vi "Save Background.vi"(8 "error in":errorcluster, 10 "File Path":path, 11 "BigMAQ in":refnum<class "BigMAQ.lvclass">) -> (0 "error out":errorcluster, 3 "BigMAQ out":refnum<class "BigMAQ.lvclass">)   [LabVIEW 2019, in "BigMAQ.lvclass"]
uses:
  BigMAQ.lvclass
  BigMAQ.lvclass/BigMAQ.ctl
  <vilib>/LabVIEW Open Source Project/Unicity/RandomStringGenerator/RandomStringGenerator.lvclass
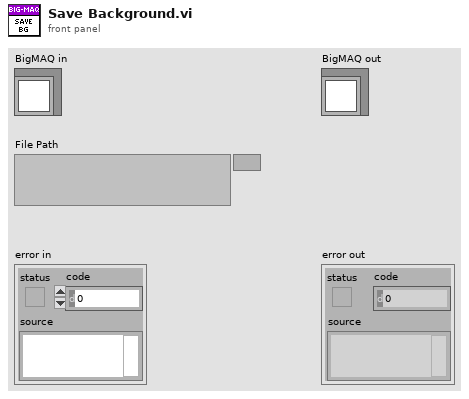
[diagram p1: front panel]
types:
  T1 = typedef "Image Type" = u32
  T2 = typedef "IMAQ Image.ctl" = refnum<image>
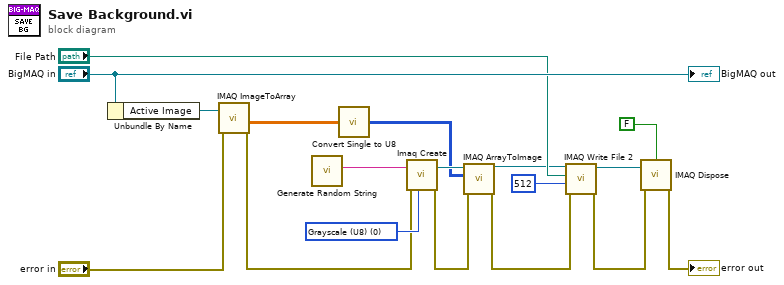
[diagram p0: block diagram]
diagram:
  w12 = T1 0 items=["Grayscale (U8)", "Grayscale (I16)", "Grayscale (SGL)", "Complex (CSG)", "RGB (U32)", "HSL (U32)", "RGB (U64)", "Grayscale (U16)"] ("Image Type")
  n1 = Unbundle By Name("BigMAQ in") -> ("Active Image"=w10:T2)
  n2 = call "IMAQ ImageToArray"("error in (no error)"="error in", "Image"=w10) -> ("Image Pixels (Float)"=w5:sgl[][], "error out"=w2:errorcluster)  [unwired: 2 in, 3 out]
  n3 = call <vilib>:"Generate Random String.vi"() -> ("Random String"=w1:string)  [unwired: 11 in]
  n4 = call "Convert Single to U8.vi"("Image Pixels (Float)"=w5) -> ("Image Pixels (U8)"=w4:u8[][])
  n5 = call "Imaq Create"("Image Name"=w1, "Image Type"=w12, "error in (no error)"=w2) -> ("New Image"=w9:T2, "error out"=w7:errorcluster)  [unwired: 2 in]
  n6 = call "IMAQ ArrayToImage"("error in (no error)"=w7, "Image Pixels (U8)"=w4, "Image"=w9) -> ("error out"=w6:errorcluster, "Image Out"=w3:T2)  [unwired: 7 in]
  n7 = call-poly "IMAQ Write File 2"("error in (no error)"=w6, "Image Quality"=u32 512, "File Path"="File Path", "Image"=w3) -> ("error out"=w11:errorcluster, "Image Out (duplicate)"=w16:T2)  [unwired: 6 in]
  n8 = call "IMAQ Dispose"("All Images? (No)"=FALSE, "Image"=w16, "error in (no error)"=w11) -> ("error out"=→"error out":errorcluster)  [unwired: 3 in]
  "BigMAQ out" <- "BigMAQ in"
